vi "test resource text utf8.vi"(8 "error in (no error)":errorcluster) -> (0 "error out":errorcluster, 3 "body":string)   [LabVIEW 2020, in "MCP Server tests.lvlib"]
doc: "resources/read of a text file must return its content as one JSON string in text. Decoded, the string must be byte for byte the UTF-8 content of the file: non-ASCII characters and line endings unchanged."
uses:
  MCP Server tests.lvlib
  <vilib>/JDP Science/JSONtext/Next JSON Value.vi
  <vilib>/JDP Science/JSONtext/String Subset.vi
  <vilib>/JDP Science/JSONtext/support/Strip Quotes and Unescape.vi
  <vilib>/JDP Science/JSONtext/Parsing/Advance past next JSON Value (inlined COPY).vi
  <vilib>/JDP Science/JSONtext/support/Unescape JSON string.vi
  <vilib>/JDP Science/JSONtext/Parsing/Advance past whitespace.vi
  <vilib>/JDP Science/JSONtext/Parsing/Advance past String.vi
  <vilib>/JDP Science/JSONtext/Parsing/Advance past Number.vi
  <vilib>/JDP Science/JSONtext/Parsing/Advance past Line Ending.vi
  <vilib>/JDP Science/JSONtext/Parsing/Parse Full Path or Item Name.vi
  <vilib>/JDP Science/JSONtext/Parsing/Advance past Array.vi
  <vilib>/JDP Science/JSONtext/Parsing/Advance past Object.vi
  <vilib>/JDP Science/JSONtext/support/Error Cluster From Code.vi
  <vilib>/JDP Science/JSONtext/Offset/Find Item Locations by Path.vi
  <vilib>/JDP Science/JSONtext/Parsing/Advance past next JSON Value.vi
  <vilib>/addons/_JKI Toolkits/Caraya/classes/Test/Test.lvclass
  <vilib>/JDP Science/JSONtext/JSONtext.lvlib
  <vilib>/addons/_JKI Toolkits/Caraya/classes/Assert/Assert.lvclass
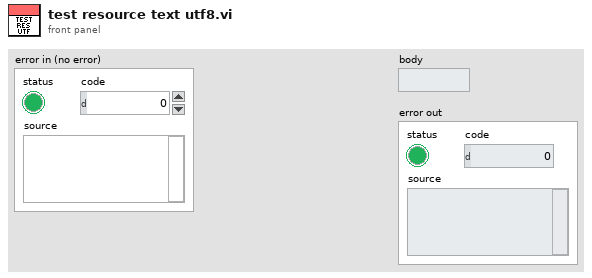
[diagram p1: front panel]
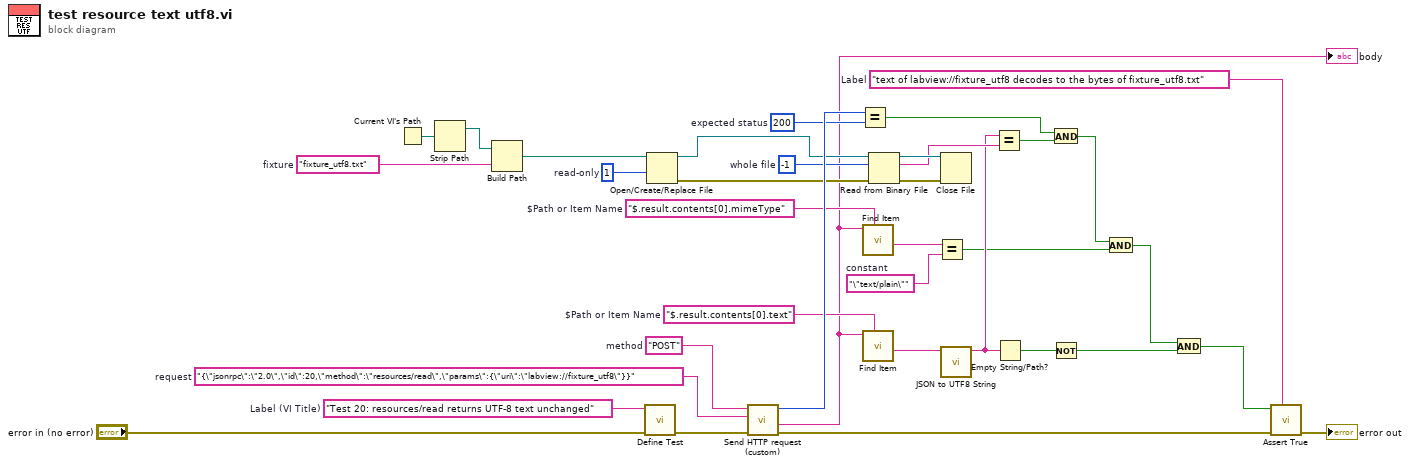
[diagram p0: block diagram]
diagram:
  w3 = "text of labview://fixture_utf8 decodes to the bytes of fixture_utf8.txt"  # Label
  w14 = "\"text/plain\""  # constant
  w20 = -1  # whole file
  w22 = u32 1  # read-only
  w24 = "fixture_utf8.txt"  # fixture
  w27 = "$.result.contents[0].mimeType"  # $Path or Item Name
  w29 = "$.result.contents[0].text"  # $Path or Item Name
  w30 = 200  # expected status
  w33 = "{\"jsonrpc\":\"2.0\",\"id\":20,\"method\":\"resources/read\",\"params\":{\"uri\":\"labview://fixture_utf8\"}}"  # request
  w34 = "POST"  # method
  w36 = "Test 20: resources/read returns UTF-8 text unchanged"  # Label (VI Title)
  n1 = Current VI's Path() -> (path=w26:path)
  n2 = Strip Path(path=w26) -> (stripped path=w25:path)  [unwired: 1 out]
  n3 = Build Path(base path=w25, name or relative path=w24) -> (appended path=w23:path)
  n4 = call <vilib>:"Define Test.vi"("error in (no error)"="error in (no error)", "Label (VI Title)"=w36) -> ("error out"=w32:errorcluster)  [unwired: 8 in, 1 out]
  n5 = Open/Create/Replace File(file path (use dialog)=w23, access (0:read/write)=w22) -> (refnum out=w21:refnum<file>, error out=w19:errorcluster)  [unwired: 4 in, 1 out]
  n6 = call "Send HTTP request (custom).vi"("error in (no error)"=w32, "request"=w33, "method"=w34) -> ("error out"=w4:errorcluster, "response"=w2:string, "status code"=w31:i32)  [unwired: 5 in, 1 out]
  "body" <- w2
  n7 = Equal?(x=w31, y=w30) -> (x = y?=w11:bool)
  n8 = call <vilib>:"Find Item.vi"("$Path or Item Name"=w27, "JSON"=w2) -> ("<JSON>"=w15:string)  [unwired: 6 in, 3 out]
  n9 = call <vilib>:"Find Item.vi"("$Path or Item Name"=w29, "JSON"=w2) -> ("<JSON>"=w28:string)  [unwired: 6 in, 3 out]
  n10 = Read from Binary File(8:w19, 10:w20, 11:w21) -> (0:w17:errorcluster, 2:w16:string, 3:w18:refnum<file>)  [unwired: 3 in, 1 out]
  n11 = Equal?(x=w15, y=w14) -> (x = y?=w8:bool)
  n12 = Close File(refnum=w18, error in=w17) -> ()  [unwired: 2 out]
  n13 = call <vilib>:"JSON to UTF8 String.vi"("JSON"=w28) -> ("<UTF8>String"=w13:string)  [unwired: 9 in, 1 out]
  n14 = Equal?(x=w13, y=w16) -> (x = y?=w10:bool)
  n15 = Empty String/Path?(string/path=w13) -> (empty?=w12:bool)
  n16 = And(x=w11, y=w10) -> (x .and. y?=w9:bool)
  n17 = Not(x=w12) -> (.not. x?=w6:bool)
  n18 = And(x=w9, y=w8) -> (x .and. y?=w7:bool)
  n19 = And(x=w7, y=w6) -> (x .and. y?=w5:bool)
  n20 = call <vilib>:"Assert True.vi"("Label"=w3, "error in (no error)"=w4, "True?"=w5) -> ("error out"=→"error out":errorcluster)  [unwired: 7 in, 1 out]
